vi "RemoteVI WS Encode Server Frame.vi"(0 "opcode":u8=2, 5 "payload":string) -> (4 "frame":string)   [LabVIEW 2020, in "RemoteVI.lvlib"]
doc: "Encodes one unmasked server-to-client WebSocket frame (RFC 6455) with FIN set: byte 0x80 OR opcode, then the payload length as 7 bits, as 126 plus a U16, or as 127 plus a U64 (big-endian), then the payload. The server never fragments. Pure function, cannot fail. Reference: encodeServerFrame() in tools\\lib\\websocket.mjs."
uses:
  RemoteVI.lvlib
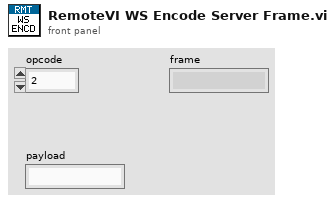
[diagram p1: front panel]
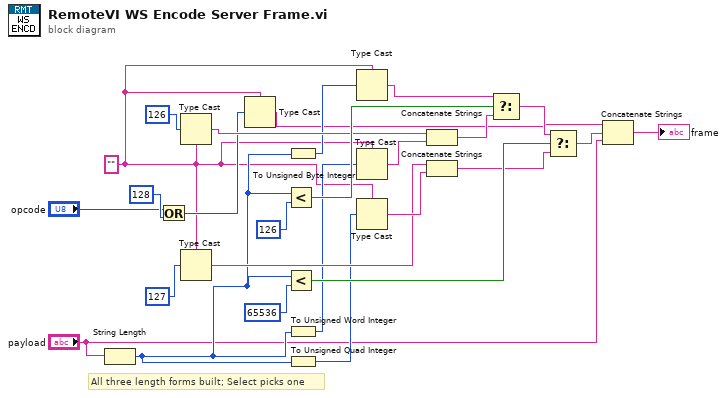
[diagram p0: block diagram]
diagram:
  w3 = ""
  # "All three length forms built; Select picks one"
  n1 = String Length(string="payload") -> (length=w11:i32)
  n2 = Or(x="opcode", y=u8 128) -> (x .or. y?=w9:u8)
  n3 = Type Cast(type=w3, x=u8 126) -> (*(type *) &x=w15:string)
  n4 = Type Cast(type=w3, x=u8 127) -> (*(type *) &x=w19:string)
  n5 = Type Cast(type=w3, x=w9) -> (*(type *) &x=w10:string)
  n6 = Less?(x=w11, y=126) -> (x < y?=w22:bool)
  n7 = Less?(x=w11, y=65536) -> (x < y?=w23:bool)
  n8 = To Unsigned Byte Integer(number=w11) -> (unsigned 8bit integer=w12:u8)
  n9 = To Unsigned Word Integer(number=w11) -> (unsigned 16bit integer=w14:u16)
  n10 = To Unsigned Quad Integer(1:w11) -> (0:w18:u64)
  n11 = Type Cast(type=w3, x=w12) -> (*(type *) &x=w13:string)
  n12 = Type Cast(type=w3, x=w14) -> (*(type *) &x=w16:string)
  n13 = Type Cast(type=w3, x=w18) -> (*(type *) &x=w20:string)
  n14 = Concatenate Strings(w15, w16) -> (w17:string)
  n15 = Concatenate Strings(w19, w20) -> (w21:string)
  n16 = Select(t=w13, s=w22, f=w17) -> (s? t:f=w24:string)
  n17 = Select(t=w24, s=w23, f=w21) -> (s? t:f=w25:string)
  n18 = Concatenate Strings(w10, w25, "payload") -> (→"frame":string)
